vi "ElevatedPass.vi"(8 "error in (no error)":errorcluster, 11 "ElevatedPassMode":T1) -> (0 "error out":errorcluster)   [LabVIEW 2013]
doc: "Automatically performs the \"Elevated Pass\" maneuver."
uses:
  ElevatedPassMode.ctl
  AnnieFramework/DoubleSolenoidAction.ctl
  AnnieFramework/RollerAction.ctl
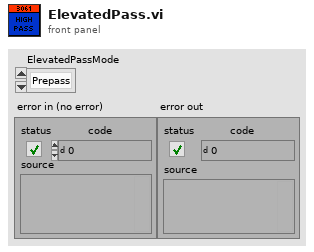
[diagram p1: front panel]
types:
  T1 = typedef "ElevatedPassMode.ctl" = enum16{"Prepass", "Pass", "Stop"}
  T2 = typedef "DoubleSolenoidAction.ctl" = enum16{"Init", "Middle", "In", "Out"}
  T3 = typedef "RollerAction.ctl" = enum16{"Init", "Off", "Forward", "Reverse"}
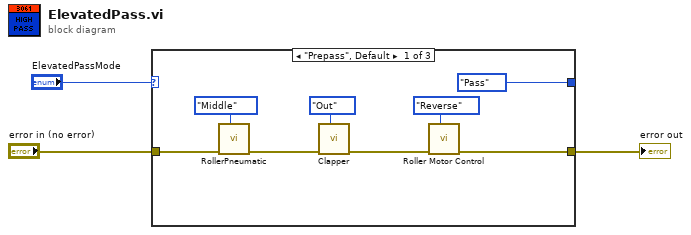
[diagram p0: block diagram]
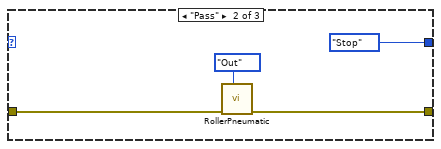
[diagram p2: hidden frame]
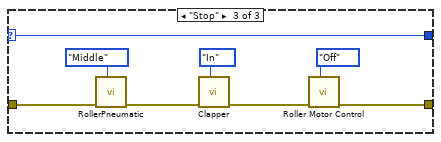
[diagram p3: hidden frame]
diagram:
  n1 = case shown="\"Prepass\", Default" "ElevatedPassMode" {
    selector: "ElevatedPassMode" -> [_ _ w16]
    tunnel: "error in (no error)" -> [w4 w14 w18]
    tunnel: [w8 w13 w17] -> w2
    tunnel: [ElevatedPassMode."Pass" ("ElevatedPassMode") ElevatedPassMode."Stop" ("ElevatedPassMode") w16] -> _
    frame "Prepass", Default {
      n2 = call "RollerPneumatic.vi"("State"=DoubleSolenoidAction."Middle", "Error in"=w4) -> ("Error out"=w5:errorcluster)  [unwired: 9 in]
      n3 = call "Clapper.vi"("State"=DoubleSolenoidAction."Out", "Error in"=w5) -> ("Error out"=w9:errorcluster)  [unwired: 9 in]
      n4 = call "Roller Motor Control.vi"("Action"=RollerAction."Reverse", "Error in"=w9) -> ("Error out"=w8:errorcluster)  [unwired: 9 in]
    }
    frame "Pass" {
      n5 = call "RollerPneumatic.vi"("State"=DoubleSolenoidAction."Out", "Error in"=w14) -> ("Error out"=w13:errorcluster)  [unwired: 9 in]
    }
    frame "Stop" {
      n6 = call "RollerPneumatic.vi"("State"=DoubleSolenoidAction."Middle", "Error in"=w18) -> ("Error out"=w19:errorcluster)  [unwired: 9 in]
      n7 = call "Clapper.vi"("State"=DoubleSolenoidAction."In", "Error in"=w19) -> ("Error out"=w20:errorcluster)  [unwired: 9 in]
      n8 = call "Roller Motor Control.vi"("Action"=RollerAction."Off", "Error in"=w20) -> ("Error out"=w17:errorcluster)  [unwired: 9 in]
    }
  }
  "error out" <- w2
